vi "Test MQTT-2.3.1-2.vi"(8 "error in (no error)":errorcluster, 11 "Connection Config":refnum<class "Connection.lvclass">) -> (0 "error out":errorcluster, 3 "Connection Config dup":refnum<class "Connection.lvclass">)   [LabVIEW 2013]
uses:
  <vilib>/LabVIEW Open Source Project/MQTT Connection/MQTT_Connection/Connection/Connection.lvclass
  <vilib>/LabVIEW Open Source Project/MQTT Control Packets/Control Packets/SUBSCRIBE/Topic Subscription -- cluster.ctl
  <vilib>/LabVIEW Open Source Project/MQTT Control Packets/Control Packets/ControlPacket/QualityOfService -- enum.ctl
  <vilib>/LabVIEW Open Source Project/MQTT Control Packets/Control Packets/ControlPacket/ControlPacket.lvclass/ControlPacket.ctl
  <vilib>/addons/_JKI Toolkits/Caraya/classes/Test/Test.lvclass
  <vilib>/addons/_JKI Toolkits/Caraya/classes/Assert/Assert.lvclass
  <vilib>/LabVIEW Open Source Project/MQTT Control Packets/Control Packets/PUBLISH/PUBLISH.lvclass
  <vilib>/LabVIEW Open Source Project/MQTT Control Packets/Control Packets/SUBSCRIBE/SUBSCRIBE.lvclass
  <vilib>/LabVIEW Open Source Project/MQTT Control Packets/Control Packets/UNSUBSCRIBE/UNSUBSCRIBE.lvclass
  <vilib>/LabVIEW Open Source Project/MQTT Control Packets/Control Packets/ControlPacket/ControlPacket.lvclass
  <vilib>/LabVIEW Open Source Project/MQTT Client/Client class/Client.lvclass
  <vilib>/LabVIEW Open Source Project/MQTT Connection/MQTT_Base/Base Class/MQTT_Base.lvclass
panel:
  out "Reserved PacketIDs":u16[](array[numeric]) format="%016b"
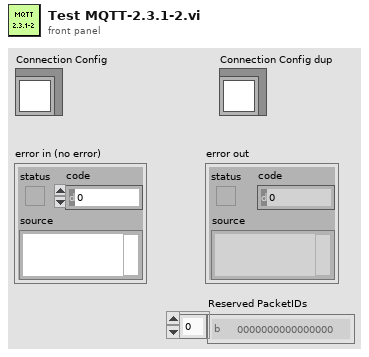
[diagram p1: front panel]
types:
  T1 = typedef "MQTT_Control_Packets.lvlib/SUBSCRIBE.lvclass/Topic Subscription -- cluster.ctl" = cluster{"Topic Filter":string, "QoS":T2}
  T2 = typedef "MQTT_Control_Packets.lvlib/ControlPacket.lvclass/QualityOfService -- enum.ctl" = enum16{"0 (At Most Once)", "1 (At Least Once)", "2 (Exactly Once)"}
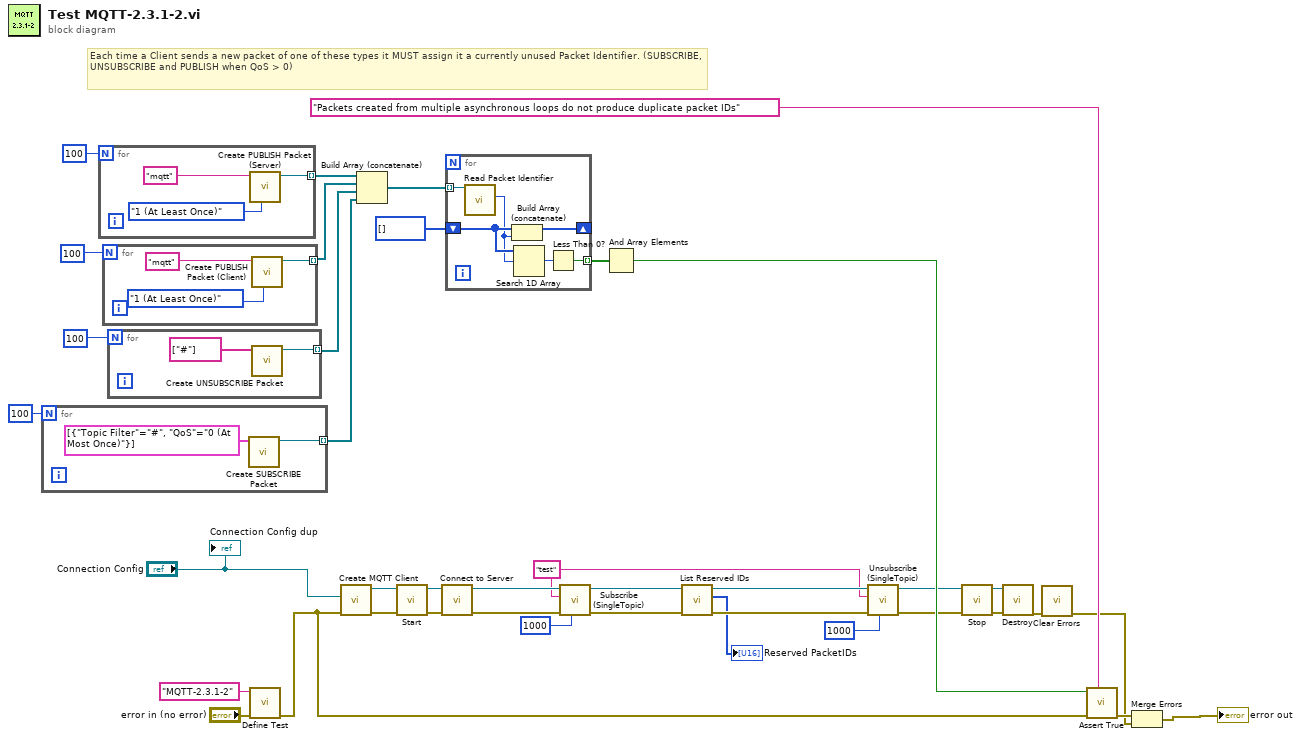
[diagram p0: block diagram]
diagram:
  w11 = "test" ("Topic Filter")
  # "Each time a Client sends a new packet of one of these types it MUST assign it a currently unused Packet Identifier. (SUBSCRIBE, UNSUBSCRIBE and PUBLISH when QoS > 0)"
  n1 = for {
    N: 100 -> [_]
    tunnel: [w41] -> w29 mode=indexing
    n2 = call <vilib>:"Create SUBSCRIBE Packet.vi"("Topic Subscriptions"=T1[] [{"Topic Filter"="#", "QoS"=enum."0 (At Most Once)"}]) -> ("SUBSCRIBE out"=w41:refnum<class "SUBSCRIBE.lvclass">)  [unwired: 8 in, 2 out]
  }
  n3 = for {
    N: 100 -> [_]
    tunnel: [w42] -> w32 mode=indexing
    n4 = call <vilib>:"Create PUBLISH Packet (Server).vi"("QoS"=QualityOfService_--_enum."1 (At Least Once)", "Topic Name"="mqtt") -> ("PUBLISH"=w42:refnum<class "PUBLISH.lvclass">)  [unwired: 6 in, 3 out]
  }
  n5 = for {
    N: 100 -> [_]
    tunnel: [w45] -> w31 mode=indexing
    n6 = call <vilib>:"Create PUBLISH Packet (Client).vi"("QoS"=QualityOfService_--_enum."1 (At Least Once)", "Topic Name"="mqtt") -> ("PUBLISH"=w45:refnum<class "PUBLISH.lvclass">)  [unwired: 6 in, 3 out]
  }
  n7 = for {
    N: 100 -> [_]
    tunnel: [w48] -> w30 mode=indexing
    n8 = call <vilib>:"Create UNSUBSCRIBE Packet.vi"("Topic Subscriptions"=string[] ["#"]) -> ("UNSUBSCRIBE out"=w48:refnum<class "UNSUBSCRIBE.lvclass">)  [unwired: 8 in, 2 out]
  }
  n9 = call <vilib>:"Define Test.vi"("error in (no error)"="error in (no error)", "Label (VI Title)"="MQTT-2.3.1-2") -> ("error out"=w3:errorcluster)  [unwired: 9 in]
  n10 = call <vilib>:"Create MQTT Client.vi"("error in (no error)"=w3, "Connection Configuration"="Connection Config") -> ("error out"=w20:errorcluster, "Client out"=w21:refnum<class "Client.lvclass">)  [unwired: 8 in]
  n11 = Build Array (concatenate)(w32, w31, w30, w29) -> (w28:refnum<class "ControlPacket.lvclass">[])
  n12 = call <vilib>:"Start.vi"("error in (no error)"=w20, "MQTT_Base in"=w21) -> ("error out"=w23:errorcluster, "MQTT_Base out"=w24:refnum<class "Client.lvclass">)  [unwired: 7 in, 1 out]
  n13 = call <vilib>:"Connect to Server.vi"("error in (no error)"=w23, "Client in"=w24) -> ("error out"=w15:errorcluster, "Client out"=w17:refnum<class "Client.lvclass">)  [unwired: 6 in, 2 out]
  n14 = for {
    tunnel: w28 -> [w55] mode=indexing
    shift-right: [w54] -> _
    shift-left: u16[] [] -> [w53]
    tunnel: [w50] -> w26 mode=indexing
    n15 = call <vilib>:"Read Packet Identifier.vi"("ControlPacket in"=w55) -> ("Packet Identifier"=w52:u16)  [unwired: 9 in, 1 out]
    n16 = Build Array (concatenate)(w53, w52) -> (w54:u16[])
    n17 = Search 1D Array(1D array=w53, element=w52) -> (index of element=w51:i32)  [unwired: 1 in]
    n18 = Less Than 0?(x=w51) -> (x < 0?=w50:bool)
  }
  n19 = call <vilib>:"Subscribe (SingleTopic).vi"("timeout (100ms)"=1000, "error in (no error)"=w15, "Topic Filter"=w11, "MQTT_Base in"=w17) -> ("error out"=w14:errorcluster, "MQTT_Base out"=w16:refnum<class "Client.lvclass">)  [unwired: 5 in, 1 out]
  n20 = And Array Elements(Boolean array=w26) -> (logical AND=w25:bool)
  n21 = call <vilib>:"List Reserved IDs.vi"("error in (no error)"=w14, "Client in"=w16) -> ("error out"=w13:errorcluster, "Reserved PacketIDs"=→"Reserved PacketIDs":u16[], "Client out"=w12:refnum<class "Client.lvclass">)  [unwired: 7 in]
  n22 = call <vilib>:"Unsubscribe (SingleTopic).vi"("timeout (100ms)"=1000, "error in (no error)"=w13, "Topic Filter"=w11, "MQTT_Base in"=w12) -> ("error out"=w9:errorcluster, "MQTT_Base out"=w10:refnum<class "Client.lvclass">)  [unwired: 5 in, 1 out]
  n23 = call <vilib>:"Stop.vi"("error in (no error)"=w9, "MQTT_Base in"=w10) -> ("error out"=w8:errorcluster, "MQTT_Base out"=w22:refnum<class "Client.lvclass">)  [unwired: 7 in, 1 out]
  n24 = call <vilib>:"Destroy.vi"("error in (no error)"=w8, "MQTT_Base in"=w22) -> ("error out"=w19:errorcluster)  [unwired: 8 in, 1 out]
  n25 = call <vilib>:"Clear Errors.vi"("error in (no error)"=w19) -> ("error out"=w1:errorcluster)  [unwired: 6 in]
  n26 = call <vilib>:"Assert True.vi"("Label"="Packets created from multiple asynchronous loops do not produce duplicate packet IDs", "error in (no error)"=w3, "True?"=w25) -> ("error out"=w18:errorcluster)  [unwired: 8 in]
  n27 = Merge Errors(w18, w1) -> (→"error out":errorcluster)
  "Connection Config dup" <- "Connection Config"
